vi "Get Supported String Tables.vi"() -> (0 "Supported Tables":T1[](array[typedef]))   [LabVIEW 2026, in "Modbus.lvlib" / "Modbus.lvclass"]
uses:
  Modbus.lvclass
  Types/Modbus Table.ctl
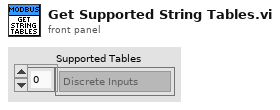
[diagram p1: front panel]
types:
  T1 = typedef "Modbus.lvlib/Modbus.lvclass/Modbus Table.ctl" = enum16{"Discrete Inputs", "Coils", "Input Registers", "Holding Registers"}
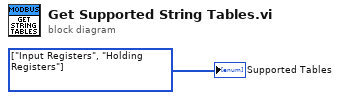
[diagram p0: block diagram]
diagram:
  w1 = T1[] [enum."Input Registers", enum."Holding Registers"] items=["Discrete Inputs", "Coils", "Input Registers", "Holding Registers"]
  "Supported Tables" <- w1
